vi "from string.vi"(8 "error in":errorcluster, 9 "data":string, 10 "version":string, 11 "CEF_Configuration in":refnum<class "CEF_serializable configuration.lvclass">) -> (0 "error out":errorcluster, 3 "CEF_Configuration out":refnum<class "CEF_serializable configuration.lvclass">)   [LabVIEW 2025, in "CEF.lvlib" / "CEF_serializable configuration.lvclass"]
doc: "Provides an interface for loading a module configuration from a file or other serialized data source. It is recommended that all children of this class store data in two sets--data required for its own initialization, and any data required for parent initialization--and that each implementation uses the <b>Call Parent Method</b> primitive to de-serialize parent information.Copyright 2017 National Instruments Corporation\n\nLicensed under the Apache License, Version 2.0 (the \"License\"); you may not use this file except in compliance with the License. You may obtain a copy of the License at http://www.apache.org/licenses/LICENSE-2.0\nUnless required by applicable law or agreed to in writing, software distributed under the License is distributed on an \"AS IS\" BASIS, WITHOUT WARRANTIES OR CONDITIONS OF ANY KIND, either express or implied. See the License for the specific language governing permissions and limitations under the License."
uses:
  CEF_serializable configuration.lvclass
  CEF_serializable configuration.lvclass/CEF_serializable configuration.ctl
  CEF.lvlib
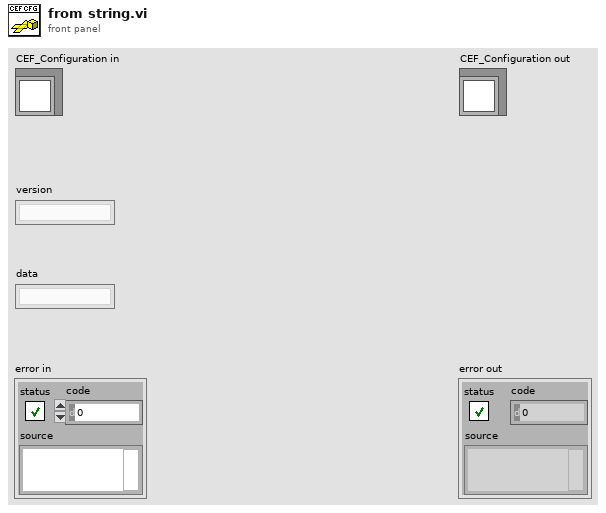
[diagram p1: front panel]
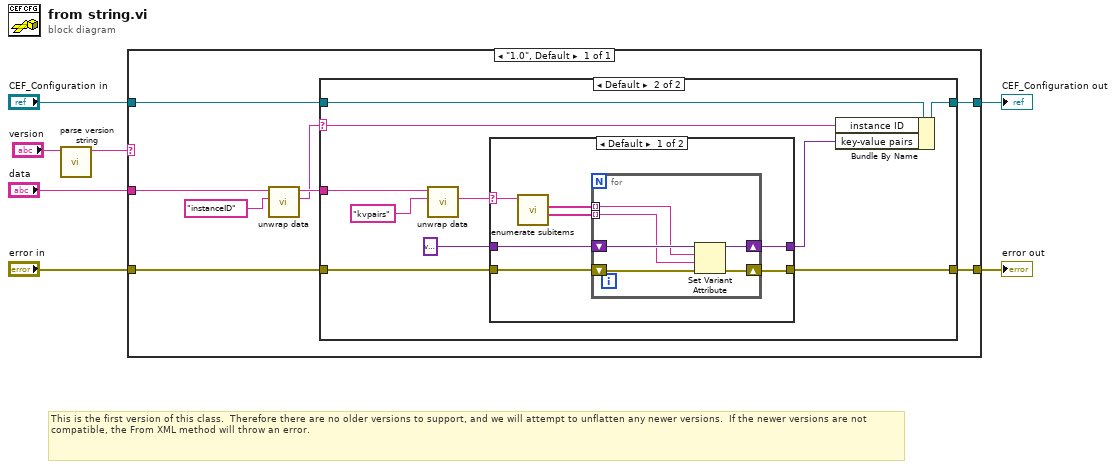
[diagram p0: block diagram]
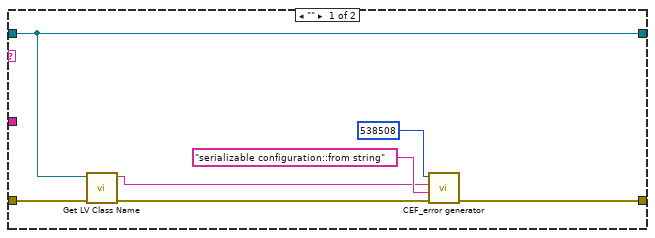
[diagram p2: hidden frame]
diagram:
  # "This is the first version of this class.  Therefore there are no older versions to support, and we will attempt to unflatten any newer versions.  If the newer versions are not compatible, the From XML method will throw an error."
  n1 = call "parse version string.vi"("full version"="version") -> ("major.minor version"=w1:string)  [unwired: 7 in, 3 out]
  n2 = case shown="\"1.0\", Default" w1 {
    tunnel: "data" -> [w13]
    tunnel: "error in" -> [w10]
    tunnel: "CEF_Configuration in" -> [w15]
    tunnel: [w14] -> w2
    tunnel: [w9] -> w3
    frame "1.0", Default {
      n3 = call "unwrap data.vi"("identifier"="instanceID" ("additional identifier"), "data to unwrap"=w13) -> ("unwrapped data"=w8:string, "remaining string"=w11:string)  [unwired: 8 in]
      n4 = case shown="Default" w8 {
        selector: w8 -> [_ w25]
        tunnel: w15 -> [w16 w32]
        tunnel: [w16 w31] -> w14
        tunnel: w11 -> [_ w30]
        tunnel: w10 -> [w19 w29]
        tunnel: [w22 w26] -> w9
        frame "" {
          n5 = call <vilib>:"Get LV Class Name.vi"("error in (no error)"=w19, "object"=w16) -> ("error out"=w18:errorcluster, "class name"=w17:string)  [unwired: 8 in]
          n6 = call "CEF_error generator.vi"("error in"=w18, "source"="serializable configuration::from string", "append error message"=w17, "error code (0)"=538508) -> ("error out"=w22:errorcluster)  [unwired: 5 in]
        }
        frame Default {
          n7 = call "unwrap data.vi"("identifier"="kvpairs" ("additional identifier"), "data to unwrap"=w30) -> ("unwrapped data"=w28:string)  [unwired: 8 in, 1 out]
          n8 = case shown="Default" w28 {
            selector: w28 -> [w37 _]
            tunnel: w29 -> [w36 w47]
            tunnel: [w39 w46] -> w27
            tunnel: [w38 w47] -> w26
            tunnel: variant ("key-value pairs") -> [w33 w46]
            frame Default {
              n9 = call "enumerate subitems.vi"("data to enumerate"=w37) -> ("associated data"=w34:string[], "discovered subitems"=w35:string[])  [unwired: 8 in, 1 out]
              n10 = for {
                shift-right: [w44] -> w39
                shift-left: w33 -> [w45]
                shift-right: [w42] -> w38
                shift-left: w36 -> [w43]
                tunnel: w35 -> [w41] mode=indexing
                tunnel: w34 -> [w40] mode=indexing
                n11 = Set Variant Attribute(Variant=w45, name=w41, value=w40, error in=w43) -> (Variant out=w44:variant, error out=w42:errorcluster)  [unwired: 1 out]
              }
            }
            frame "" {
            }
          }
          n12 = Bundle By Name(cluster=w32, "instance ID"=w25, "key-value pairs"=w27) -> (w31:refnum<class "CEF_serializable configuration.lvclass">)
        }
      }
    }
  }
  "error out" <- w3
  "CEF_Configuration out" <- w2
